vi "Call Revert to Scan Mode.vi"(8 "error in":errorcluster, 10 "Target IP Address":string, 11 "Slave Ref":string) -> (0 "error out":errorcluster)   [LabVIEW 2027, in "SEECD System Explorer.lvlib"]
uses:
  SEECD System Explorer.lvlib
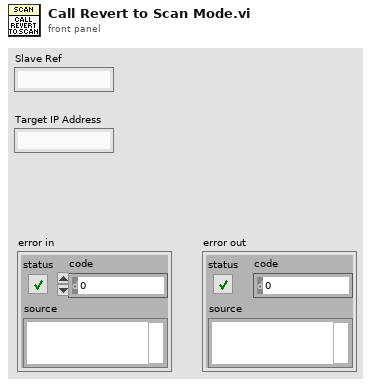
[diagram p1: front panel]
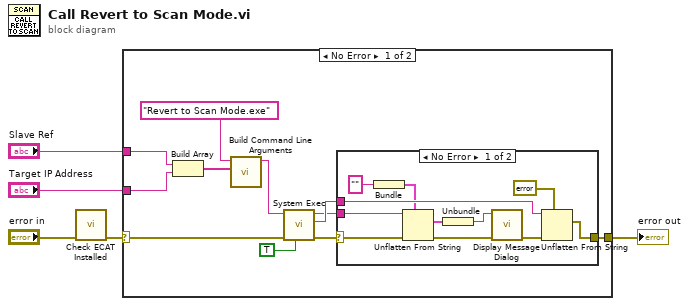
[diagram p0: block diagram]
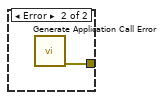
[diagram p2: hidden frame]
diagram:
  n1 = call "Check ECAT Installed.vi"("error in"="error in") -> ("error out"=w1:errorcluster)  [unwired: 10 in]
  n2 = case shown="No Error" w1 {
    selector: w1 -> [w16 w29]
    tunnel: [w14 w29] -> w3
    tunnel: "Slave Ref" -> [w10 _]
    tunnel: "Target IP Address" -> [w9 _]
    frame No Error {
      n3 = Build Array(w10, w9) -> (w8:string[])
      n4 = call "Build Command Line Arguments.vi"("Arguments"=w8, "Executable File Name"="Revert to Scan Mode.exe" ("name or relative path")) -> ("Command Line"=w7:string)  [unwired: 9 in]
      n5 = call <vilib>:"System Exec.vi"("run minimized? (F)"=TRUE, "error in (no error)"=w16, "command line"=w7) -> ("error out"=w15:errorcluster, "standard error"=w13:string, "standard output"=w6:string)  [unwired: 5 in, 1 out]
      n6 = case shown="No Error" w15 {
        selector: w15 -> [w23 _]
        tunnel: [w26 w28] -> w14
        tunnel: w13 -> [w25 _]
        tunnel: w6 -> [w20 _]
        frame No Error {
          n7 = Bundle("") -> (w21:cluster{string})  [unwired: 1 in]
          n8 = Unflatten From String(type=w21, binary string=w20, error in (no error)=w23) -> (value=w18:cluster{string}, error out=w22:errorcluster)  [unwired: 2 in, 1 out]
          n9 = Unbundle(w18) -> (w17:string)
          n10 = call "Display Message Dialog.vi"("error in"=w22, "Message to display"=w17) -> ("error out"=w24:errorcluster)  [unwired: 9 in]
          n11 = Unflatten From String(type=errorcluster {"status"=FALSE, "code"=0, "source"=""} ("error in (no error)"), binary string=w25, error in (no error)=w24) -> (value=w26:errorcluster)  [unwired: 2 in, 2 out]
        }
        frame Error {
          n12 = call "Generate Application Call Error.vi"() -> ("error out"=w28:errorcluster)  [unwired: 11 in]
        }
      }
    }
    frame Error {
    }
  }
  "error out" <- w3
